vi "Measurement Logic.vi"() -> ()   [LabVIEW 2022 SP3, in "Generation_Class D Amplifier.lvlib"]
uses:
  Generation_Class D Amplifier.lvlib
  service/generation/API/AudioGeneration/AudioGeneration.lvclass
  Measurement Results.ctl
  shared/digital serial gen settings/digital audio protocol controls.lvlib
  shared/analog gen settings/Analog Gen Settings.lvlib
  service/generation/API/AudioGeneration/Configure - Digital.vi
  service/generation/API/AudioGeneration/Configure - Analog.vi
  service/generation/controls/generation type.ctl
  service/generation/controls/AudioGenTypeDefs.lvlib
  service/generation/controls/signal type.ctl
  service/generation/controls/signal settings.ctl
  shared/controls/digital output level units.ctl
  shared/controls/audio controls.lvlib
  Measurement Configuration.ctl
  generation control.ctl
  shared/controls/generation type.ctl
  <vilib>/Plug-In SDKs/Measurements/Measure Call Context/Measure Call Context.lvclass
panel:
  out "measure call context out":refnum<class "Measure Call Context.lvclass">
  in  "measure call context in":refnum<class "Measure Call Context.lvclass">
  out "measurement results":T1
  in  "measurement configuration":T2={"digital channel list"="7821\\PCMo 8", "master clock channel list"="7821\\PCMo 0", "output level units"=enum."% FS", "generation control"=enum."Stop", "output configuration file"="", "generation type"=enum."Analog", "analog output channel"="", "signal parameters"=""}
  out "error out":errorcluster
  in  "error in":errorcluster
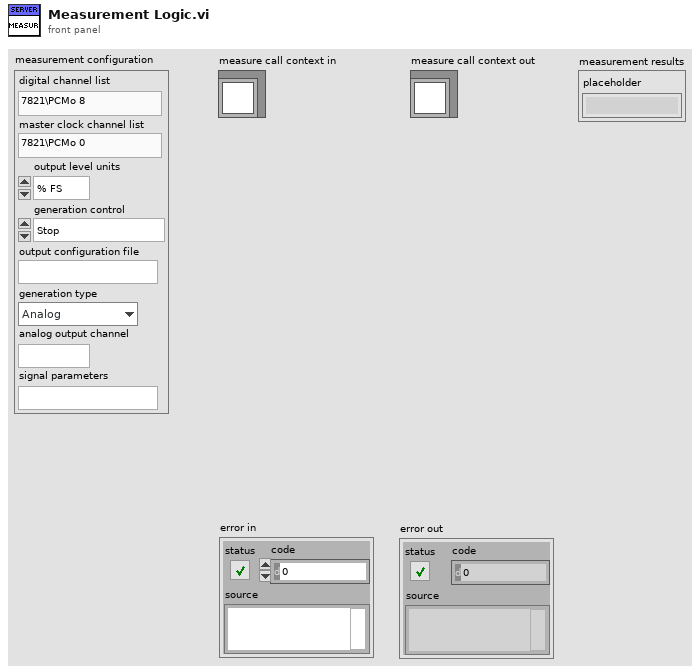
[diagram p1: front panel]
types:
  T1 = typedef "Generation_Class D Amplifier.lvlib/Measurement Results.ctl" = cluster{"placeholder":string}
  T2 = typedef "Generation_Class D Amplifier.lvlib/Measurement Configuration.ctl" = cluster{"digital channel list":string, "master clock channel list":string, "output level units":T3, "generation control":T4, "output configuration file":string, "generation type":T5, "analog output channel":string, "signal parameters":string}
  T3 = typedef "audio controls.lvlib/digital output level units.ctl" = enum32{"% FS", "dBFS", "V"}
  T4 = typedef "Generation_Class D Amplifier.lvlib/generation control.ctl" = enum32{"Start", "Stop"}
  T5 = typedef "generation type.ctl" = enum32{"Analog", "Digital Serial"}
  T6 = typedef "AudioGenTypeDefs.lvlib/generation type.ctl" = enum16{"analog", "digital"}
  T7 = typedef "AudioGenTypeDefs.lvlib/signal type.ctl" = enum16{"Sine", "Dual Tone"}
  T8 = typedef "AudioGenTypeDefs.lvlib/signal settings.ctl" = cluster{"signal type":T7, "properties":string, "output level units":T3}
  T9 = typedef "AudioGenTypeDefs.lvlib/generation status.ctl" = enum16{"Idle", "Committed", "Active"}
  T10 = typedef "AudioGenTypeDefs.lvlib/analog output settings.ctl" = cluster{"output rate":dbl, "range":dbl, "terminal configuration":T11, "output impedance":dbl, "common mode offset":dbl, "pure tone mode":bool}
  T11 = typedef "AudioGenTypeDefs.lvlib/terminal configuration.ctl" = enum32{"Default", "RSE", "Differential", "Pseudodifferential"}
  T12 = typedef "digital serial gen settings.ctl" = cluster{"number of channels":u32, "data justification":T13, "endianness":T14, "channel length":u32, "bit depth":u32, "frame clock rate":dbl, "bit clock edge sync":T15, "master clock rate":dbl, "Logic Level":T16, "frame sync edge for channel 0":T15, "Channel 0 Offset":u32}
  T13 = typedef "PDM Shared.lvlib/PCM Data Justification.ctl" = enum16{"Left Justified", "Right Justified"}
  T14 = typedef "PDM Shared.lvlib/PCM Bit Endianness.ctl" = enum16{"MSB First", "LSB First"}
  T15 = typedef "PDM Shared.lvlib/Digital Edge.ctl" = enum8{"Rising", "Falling"}
  T16 = typedef "PDM Acquisition Class Library.lvlib/DecoderSession.lvclass/Logic Levels.ctl" = enum16{"3.3 V", "1.8 V", "1.2 V"}
  T17 = typedef "AudioGenTypeDefs.lvlib/digital protocol settings.ctl" = cluster{"logic level":T16, "PCM Data Configuration":T18, "bit clock rate":sgl, "master clock rate":sgl, "clock mode":T19, "Frame Sync Clock Control":T20}
  T18 = typedef "PDM Shared.lvlib/PCM Data Format Configuration.ctl" = cluster{"Frame Sync Edge for Channel 0":T15, "Channel Count Per Frame":u8, "Channel Length":u16, "Bit Depth":u8, "Channel 0 Offset":u16, "Endianness":T14, "Data Justification":T13}
  T19 = typedef "PDM Shared.lvlib/clock mode.ctl" = enum16{"divided clock", "DDS"}
  T20 = typedef "PDM Shared.lvlib/PCM Frame Sync Control.ctl" = cluster{"Frame Length":u16, "Frame Sync Pulse Width":u16, "Bit Clock Edge  Sync":T15}
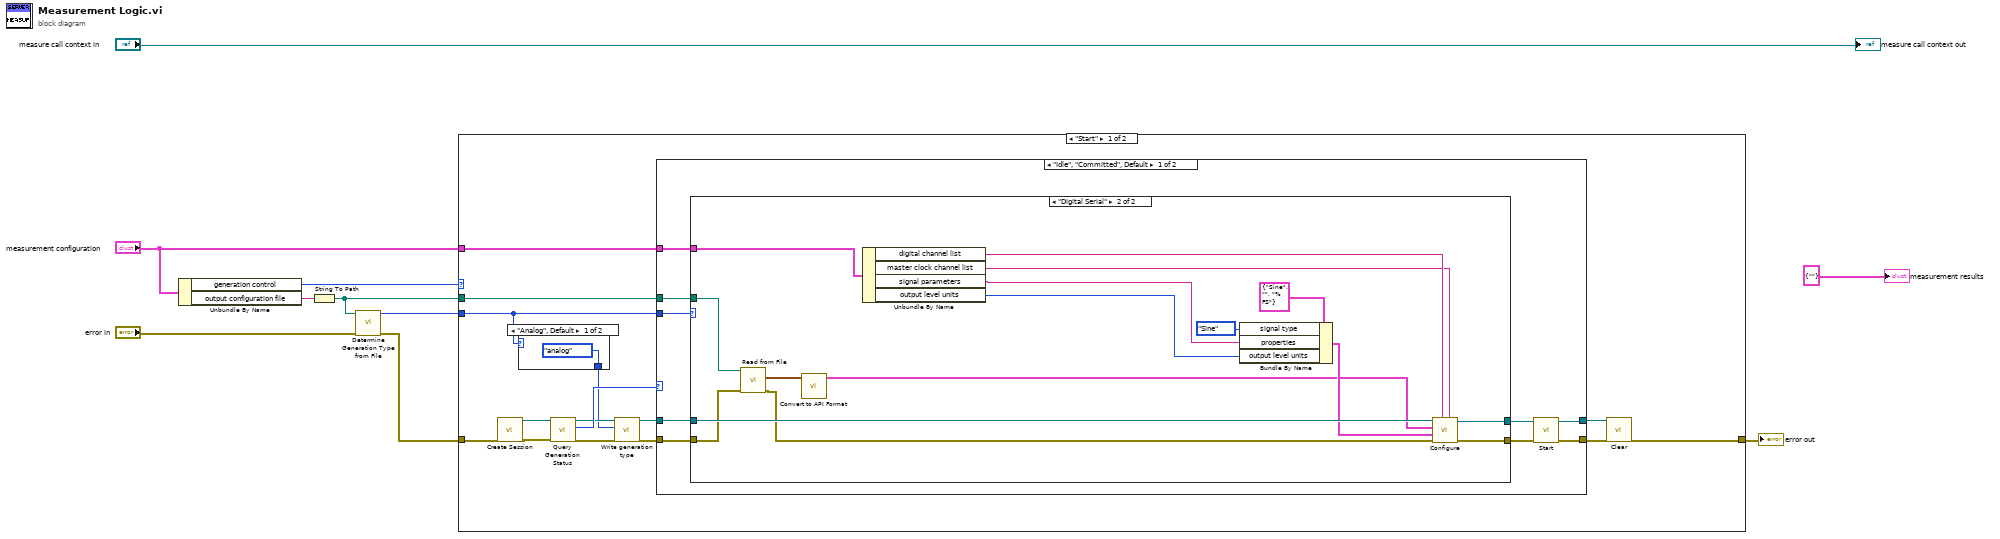
[diagram p0: block diagram]
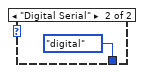
[diagram p2: hidden frame]
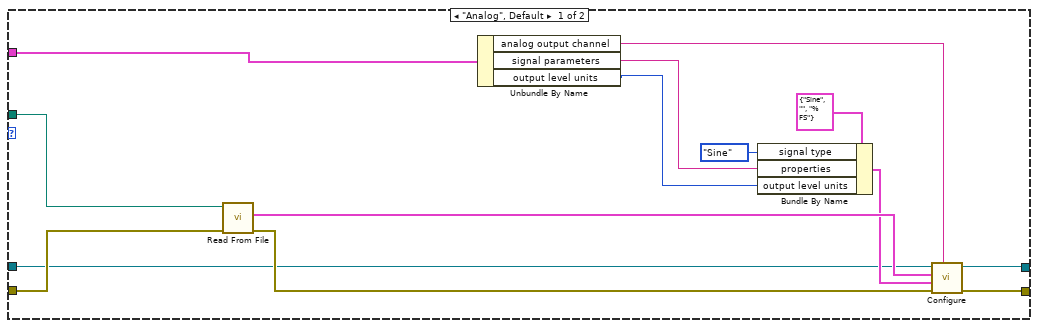
[diagram p3: hidden frame]
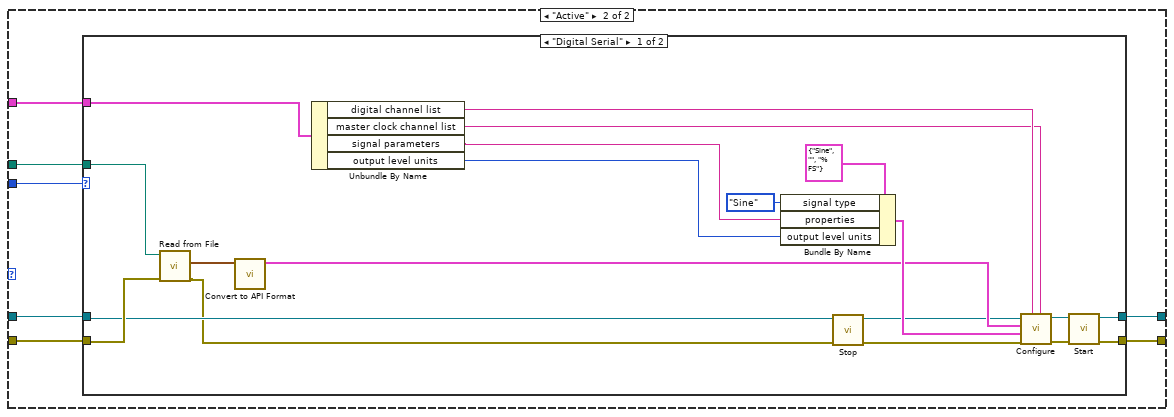
[diagram p4: hidden frame]
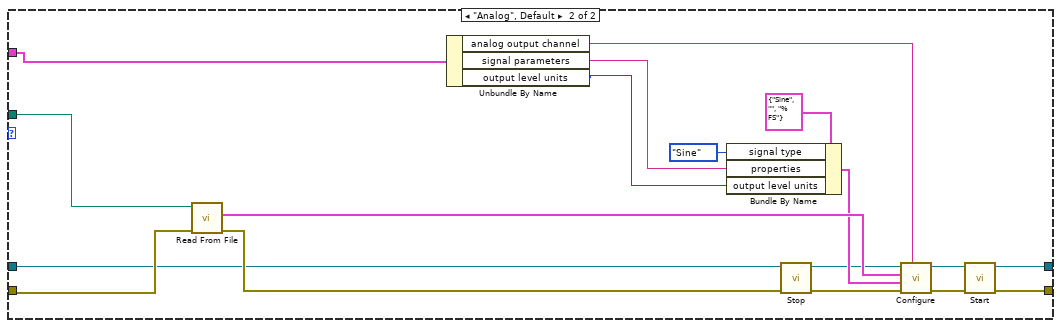
[diagram p5: hidden frame]
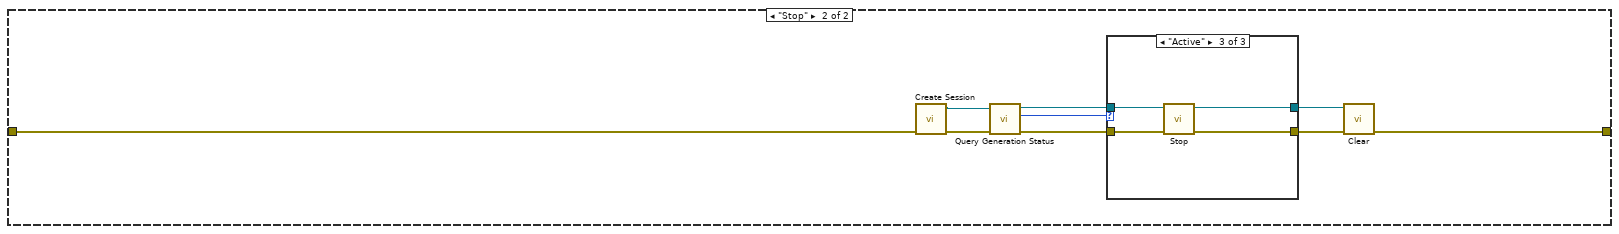
[diagram p6: hidden frame]
diagram:
  n1 = Unbundle By Name("measurement configuration") -> ("generation control"=w8:T4, "output configuration file"=w6:string)
  n2 = String To Path(string=w6) -> (path=w2:path)
  n3 = call "Determine Generation Type from File.vi"("error in (no error)"="error in", "cfg file"=w2) -> ("error out"=w3:errorcluster, "output type"=w4:T5)  [unwired: 8 in]
  n4 = case shown="\"Start\"" w8 {
    tunnel: w3 -> [w24 w115]
    tunnel: [w23 w114] -> w9
    tunnel: w4 -> [w12 _]
    tunnel: w2 -> [w18 _]
    tunnel: "measurement configuration" -> [w17 _]
    frame "Start" {
      n5 = call "Create Session.vi"("error in (no error)"=w24) -> ("error out"=w19:errorcluster, "session out"=w20:refnum<class "AudioGeneration.lvclass">)  [unwired: 9 in]
      n6 = case shown="\"Analog\", Default" w12 {
        tunnel: [generation_type."analog" ("generation type") generation_type."digital" ("generation type")] -> w11
        frame "Analog", Default {
        }
        frame "Digital Serial" {
        }
      }
      n7 = call "Query Generation Status.vi"("error in (no error)"=w19, "AudioGeneration in"=w20) -> ("error out"=w16:errorcluster, "status"=w25:T9, "AudioGeneration out"=w15:refnum<class "AudioGeneration.lvclass">)  [unwired: 5 in, 2 out]
      n8 = call-dynamic "Write generation type.vi"("error in (no error)"=w16, "generation type"=w11, "AudioGeneration in"=w15) -> ("error out"=w13:errorcluster, "AudioGeneration out"=w14:refnum<class "AudioGeneration.lvclass">)  [unwired: 7 in]
      n9 = case shown="\"Idle\", \"Committed\", Default" w25 {
        tunnel: w14 -> [w34 w73]
        tunnel: w13 -> [w33 w71]
        tunnel: [w32 w72] -> w22
        tunnel: [w31 w70] -> w21
        tunnel: w12 -> [w30 w69]
        tunnel: w18 -> [w29 w67]
        tunnel: w17 -> [w28 w68]
        frame "Idle", "Committed", Default {
          n10 = case shown="\"Digital Serial\"" w30 {
            tunnel: [w50 w66] -> w36
            tunnel: [w49 w65] -> w35
            tunnel: w34 -> [w38 w64]
            tunnel: w33 -> [w48 w62]
            tunnel: w29 -> [w47 w61]
            tunnel: w28 -> [w46 w59]
            frame "Analog", Default {
              n11 = call "Read From File.vi"("error in (no error)"=w48, "file path"=w47) -> ("error out"=w39:errorcluster, "analog generation"=w44:T10)  [unwired: 7 in, 1 out]
              n12 = Unbundle By Name(w46) -> ("analog output channel"=w45:string, "signal parameters"=w41:string, "output level units"=w37:T3)
              n13 = Bundle By Name(cluster=T8 {"signal type"=enum."Sine", "properties"="", "output level units"=enum."% FS"} ("signal settings"), "signal type"=signal_type."Sine", "properties"=w41, "output level units"=w37) -> (w40:T8)
              n14 = call-poly "Configure.vi"("DAQmx Physical Channel"=w45, "error in (no error)"=w39, "signal settings"=w40, "output settings"=w44, "AudioGeneration in"=w38) -> ("error out"=w49:errorcluster, "AudioGeneration out"=w50:refnum<class "AudioGeneration.lvclass">)  [unwired: 5 in]
            }
            frame "Digital Serial" {
              n15 = call "Read from File.vi"("error in (no error)"=w62, "file path"=w61) -> ("error out"=w60:errorcluster, "digital audio protocol settings"=w63:T12)  [unwired: 7 in, 1 out]
              n16 = call "Convert to API Format.vi"("digital audio protocol settings"=w63) -> ("digital protocol settings"=w52:T17)  [unwired: 10 in]
              n17 = Unbundle By Name(w59) -> ("digital channel list"=w58:string, "master clock channel list"=w57:string, "signal parameters"=w53:string, "output level units"=w51:T3)
              n18 = Bundle By Name(cluster=T8 {"signal type"=enum."Sine", "properties"="", "output level units"=enum."% FS"} ("signal settings"), "signal type"=signal_type."Sine", "properties"=w53, "output level units"=w51) -> (w55:T8)
              n19 = call-poly "Configure.vi"("master clock channel list"=w57, "data channel list"=w58, "error in (no error)"=w60, "signal settings"=w55, "digital protocol settings"=w52, "AudioGeneration in"=w64) -> ("error out"=w65:errorcluster, "AudioGeneration out"=w66:refnum<class "AudioGeneration.lvclass">)  [unwired: 4 in]
            }
          }
          n20 = call "Start.vi"("error in (no error)"=w35, "AudioGeneration in"=w36) -> ("error out"=w31:errorcluster, "AudioGeneration out"=w32:refnum<class "AudioGeneration.lvclass">)  [unwired: 8 in]
        }
        frame "Active" {
          n21 = case shown="\"Digital Serial\"" w69 {
            tunnel: w73 -> [w75 w94]
            tunnel: [w83 w102] -> w72
            tunnel: w71 -> [w80 w98]
            tunnel: [w82 w101] -> w70
            tunnel: w68 -> [w78 w100]
            tunnel: w67 -> [w79 w99]
            frame "Digital Serial" {
              n22 = call "Read from File.vi"("error in (no error)"=w80, "file path"=w79) -> ("error out"=w74:errorcluster, "digital audio protocol settings"=w93:T12)  [unwired: 7 in, 1 out]
              n23 = call "Convert to API Format.vi"("digital audio protocol settings"=w93) -> ("digital protocol settings"=w86:T17)  [unwired: 10 in]
              n24 = Unbundle By Name(w78) -> ("digital channel list"=w92:string, "master clock channel list"=w91:string, "signal parameters"=w87:string, "output level units"=w85:T3)
              n25 = Bundle By Name(cluster=T8 {"signal type"=enum."Sine", "properties"="", "output level units"=enum."% FS"} ("signal settings"), "signal type"=signal_type."Sine", "properties"=w87, "output level units"=w85) -> (w89:T8)
              n26 = call "Stop.vi"("error in (no error)"=w74, "AudioGeneration in"=w75) -> ("error out"=w76:errorcluster, "AudioGeneration out"=w77:refnum<class "AudioGeneration.lvclass">)  [unwired: 8 in]
              n27 = call-poly "Configure.vi"("master clock channel list"=w91, "data channel list"=w92, "error in (no error)"=w76, "signal settings"=w89, "digital protocol settings"=w86, "AudioGeneration in"=w77) -> ("error out"=w81:errorcluster, "AudioGeneration out"=w84:refnum<class "AudioGeneration.lvclass">)  [unwired: 4 in]
              n28 = call "Start.vi"("error in (no error)"=w81, "AudioGeneration in"=w84) -> ("error out"=w82:errorcluster, "AudioGeneration out"=w83:refnum<class "AudioGeneration.lvclass">)  [unwired: 8 in]
            }
            frame "Analog", Default {
              n29 = call "Read From File.vi"("error in (no error)"=w98, "file path"=w99) -> ("error out"=w95:errorcluster, "analog generation"=w110:T10)  [unwired: 7 in, 1 out]
              n30 = Unbundle By Name(w100) -> ("analog output channel"=w111:string, "signal parameters"=w107:string, "output level units"=w105:T3)
              n31 = Bundle By Name(cluster=T8 {"signal type"=enum."Sine", "properties"="", "output level units"=enum."% FS"} ("signal settings"), "signal type"=signal_type."Sine", "properties"=w107, "output level units"=w105) -> (w106:T8)
              n32 = call "Stop.vi"("error in (no error)"=w95, "AudioGeneration in"=w94) -> ("error out"=w96:errorcluster, "AudioGeneration out"=w97:refnum<class "AudioGeneration.lvclass">)  [unwired: 8 in]
              n33 = call-poly "Configure.vi"("DAQmx Physical Channel"=w111, "error in (no error)"=w96, "signal settings"=w106, "output settings"=w110, "AudioGeneration in"=w97) -> ("error out"=w103:errorcluster, "AudioGeneration out"=w104:refnum<class "AudioGeneration.lvclass">)  [unwired: 5 in]
              n34 = call "Start.vi"("error in (no error)"=w103, "AudioGeneration in"=w104) -> ("error out"=w101:errorcluster, "AudioGeneration out"=w102:refnum<class "AudioGeneration.lvclass">)  [unwired: 8 in]
            }
          }
        }
      }
      n35 = call "Clear.vi"("error in (no error)"=w21, "AudioGeneration in"=w22) -> ("error out"=w23:errorcluster)  [unwired: 9 in]
    }
    frame "Stop" {
      n36 = call "Create Session.vi"("error in (no error)"=w115) -> ("error out"=w112:errorcluster, "session out"=w113:refnum<class "AudioGeneration.lvclass">)  [unwired: 9 in]
      n37 = call "Query Generation Status.vi"("error in (no error)"=w112, "AudioGeneration in"=w113) -> ("error out"=w118:errorcluster, "status"=w120:T9, "AudioGeneration out"=w119:refnum<class "AudioGeneration.lvclass">)  [unwired: 5 in, 2 out]
      n38 = case shown="\"Active\"" w120 {
        tunnel: w119 -> [w122 w124 w128]
        tunnel: w118 -> [w121 w123 w127]
        tunnel: [w122 w124 w126] -> w117
        tunnel: [w121 w123 w125] -> w116
        frame "Idle", Default {
        }
        frame "Committed" {
        }
        frame "Active" {
          n39 = call "Stop.vi"("error in (no error)"=w127, "AudioGeneration in"=w128) -> ("error out"=w125:errorcluster, "AudioGeneration out"=w126:refnum<class "AudioGeneration.lvclass">)  [unwired: 8 in]
        }
      }
      n40 = call "Clear.vi"("error in (no error)"=w116, "AudioGeneration in"=w117) -> ("error out"=w114:errorcluster)  [unwired: 9 in]
    }
  }
  "error out" <- w9
  "measurement results" <- T1 {"placeholder"=""} ("measurement results")
  "measure call context out" <- "measure call context in"
